vi "Reflection Native Invoke Method.vi"(8 "error in (no error)":errorcluster, 9 "parameters":refnum<k24>[](array[refnum]), 10 "Target Object":refnum<k24>, 11 "Method Info in":refnum<k24>) -> (0 "error out":errorcluster, 2 "Return Value":refnum<k24>, 3 "Method Info out":refnum<k24>)   [LabVIEW 2026, in "ToastNotification.lvlib" / "Reflection DotNet.lvlib"]
doc: "Native MethodInfo.Invoke call using Target Object and parameters. Borrow the Method Info and argument handles. Return Value is an acquired boxed result, which the caller closes even on failure; void methods may return null. An unwired parameters array is empty for parameterless methods. Method Info out aliases the input metadata."
uses:
  Reflection DotNet.lvlib
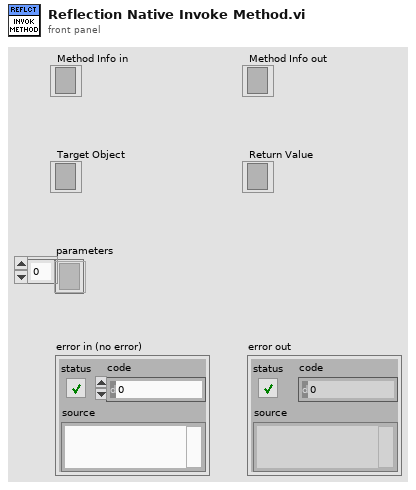
[diagram p1: front panel]
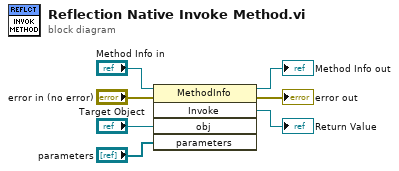
[diagram p0: block diagram]
diagram:
  n1 = invoke class="MethodInfo" method="Invoke"(reference="Method Info in", error in="error in (no error)", "obj"="Target Object", "parameters"="parameters") -> (reference out=→"Method Info out":refnum<k24>, error out=→"error out":errorcluster, "Invoke"=→"Return Value":refnum<k24>)  [unwired: 1 in, 2 out]
